vi "VIH - CHM Project - Check Environment.vi"(8 "error in":errorcluster) -> (0 "error out":errorcluster, 2 "HHC path":path, 3 "Flags":T1, 4 "Download URL":string)   [LabVIEW 2014]
doc: "::: VI Helpeks :::\nCopyright (c) 2000-2026 Konstantin Shifershteyn. All rights reserved."
panel:
  # "VI Helpeks\nCopyright (c) 2012-2026 Konstantin Shifershteyn"
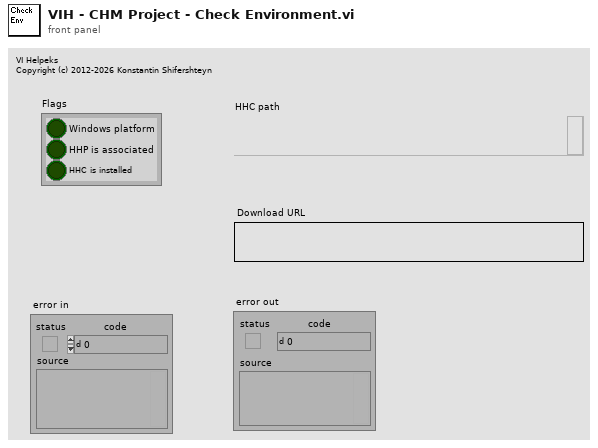
[diagram p1: front panel]
types:
  T1 = cluster{"Windows platform":bool, "HHP is associated":bool, "HHC is installed":bool}
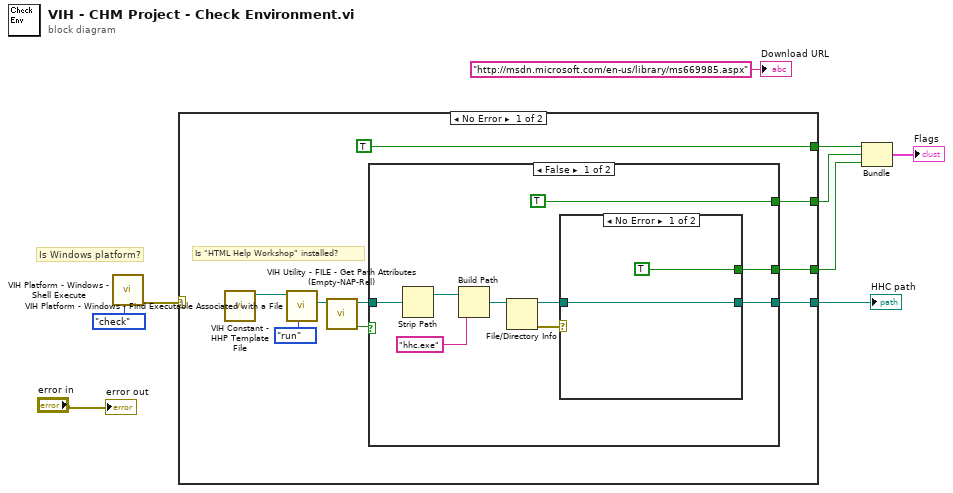
[diagram p0: block diagram]
diagram:
  # "Is Windows platform?"
  n1 = call "VIH Platform - Windows - Shell Execute.vi"("cmd (run)"=enum16{"run", "check"}."check") -> ("error out"=w8:errorcluster)  [unwired: 10 in]
  n2 = case shown="No Error" w8 {
    tunnel: [TRUE _] -> w5
    tunnel: [w13 _] -> w4
    tunnel: [w11 _] -> w7
    tunnel: [w10 _] -> w3
    frame No Error {
      # "Is \"HTML Help Workshop\" installed?"
      n3 = call "VIH Constant - HHP Template File.vi"() -> ("HHP Template File path"=w17:path)  [unwired: 11 in]
      n4 = call "VIH Platform - Windows - Find Executable Associated with a File.vi"("cmd (run)"=enum16{"run", "check"}."run", "Document path"=w17) -> ("ExePath"=w18:path)  [unwired: 8 in, 1 out]
      n5 = call "VIH Utility - FILE - Get Path Attributes (Empty-NAP-Rel).vi"("Path"=w18) -> ("Not A Path or Empty path"=w14:bool, "dup Path"=w12:path)  [unwired: 6 in, 3 out]
      n6 = case shown="False" w14 {
        tunnel: [TRUE _] -> w13
        tunnel: w12 -> [w26 _]
        tunnel: [w21 _] -> w11
        tunnel: [w19 _] -> w10
        frame False {
          n7 = Strip Path(path=w26) -> (stripped path=w25:path)  [unwired: 1 out]
          n8 = Build Path(base path=w25, name or relative path="hhc.exe") -> (appended path=w23:path)
          n9 = File/Directory Info(path=w23) -> (path out=w20:path, error out=w22:errorcluster)  [unwired: 1 in, 5 out]
          n10 = case shown="No Error" w22 {
            tunnel: [w29 _] -> w21
            tunnel: w20 -> [w29 _]
            tunnel: [TRUE _] -> w19
            frame No Error {
            }
            frame Error {
            }
          }
        }
        frame True {
        }
      }
    }
    frame Error {
    }
  }
  "HHC path" <- w7
  n11 = Bundle(w5, w4, w3) -> (→"Flags":cluster{bool, bool, bool})  [unwired: 1 in]
  "error out" <- "error in"
  "Download URL" <- "http://msdn.microsoft.com/en-us/library/ms669985.aspx" ("Download URL")
